vi "Test is String Constant a State Constant.vi"(8 "error in (no error)":errorcluster) -> (0 "error out":errorcluster)   [LabVIEW 2020, in "TEST JKI State Machine API.lvlib"]
uses:
  TEST JKI State Machine API.lvlib
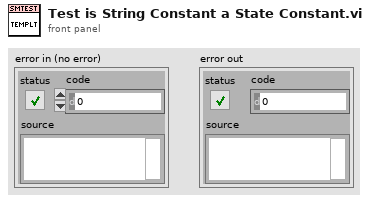
[diagram p1: front panel]
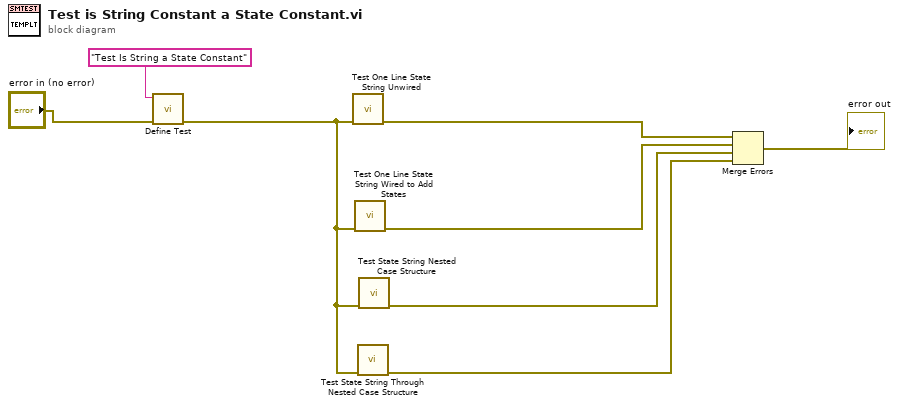
[diagram p0: block diagram]
diagram:
  n1 = call <vilib>:"Define Test.vi"("error in (no error)"="error in (no error)", "Label (VI Title)"="Test Is String a State Constant") -> ("error out"=w3:errorcluster)  [unwired: 8 in, 1 out]
  n2 = call "Test One Line State String Unwired.vi"("error in (no error)"=w3) -> ("error out"=w4:errorcluster)  [unwired: 10 in]
  n3 = call "Test One Line State String Wired to Add States.vi"("error in (no error)"=w3) -> ("error out"=w6:errorcluster)  [unwired: 10 in]
  n4 = call "Test State String Through Nested Case Structure.vi"("error in (no error)"=w3) -> ("error out"=w1:errorcluster)  [unwired: 10 in]
  n5 = call "Test State String Nested Case Structure.vi"("error in (no error)"=w3) -> ("error out"=w2:errorcluster)  [unwired: 10 in]
  n6 = Merge Errors(w4, w6, w2, w1) -> (→"error out":errorcluster)
